vi "Registry-Based Logging (Wireless).vi"() -> ()   [LabVIEW 2018]
uses:
  api/logger_class/Log Levels.ctl
  api/logger_class/Failure Information.ctl
  api/logger_class/Log Record.ctl
  api/logger_class/Internal Log Levels.ctl
  ff44e4a9-c346-414c-ae2a-efcf3ff82913.vi
  968e9200-95f1-4d5c-ab7a-f172df11adbb.vi
  5746b3ac-eb64-4ad0-8e88-1d5da43a9e78.vi
  ee222f89-d58e-4e28-8b53-aa2841b98c47.vi
  645936a5-18e5-41ae-9078-b5e4c552694f.vi
  c7798b5a-73a1-416c-972e-a12d59322e34.vi
  1f8b4f84-eef8-41cb-aaa5-2323aa4fe3ca.vi
  b5f8ac20-1bad-4c30-9ea3-a10bb6eeb7f6.vi
  968e9200-95f1-4d5c-ab7a-f172df11adbb.vi/caf2d4a3-5a7b-40e1-b7b0-74b52901b9f9.vi
  5746b3ac-eb64-4ad0-8e88-1d5da43a9e78.vi/a02c6254-97f5-44e3-a3a9-7fdb6dfbd055.vi
  ee222f89-d58e-4e28-8b53-aa2841b98c47.vi/bae24b8d-f663-491e-8374-2218e527d0d0.vi
  api/Log.vi
  645936a5-18e5-41ae-9078-b5e4c552694f.vi/bf655d3c-1ce4-400f-a78f-0f3f0191886e.vi
  api/Mark Error.vi
  c7798b5a-73a1-416c-972e-a12d59322e34.vi/ba94d47b-0e30-4c32-b8ff-86d609cd95a5.vi
  968e9200-95f1-4d5c-ab7a-f172df11adbb.vi/caf2d4a3-5a7b-40e1-b7b0-74b52901b9f9.vi/0a1ee2ab-da6d-4243-8cf3-8125e611a602.vi
  5746b3ac-eb64-4ad0-8e88-1d5da43a9e78.vi/a02c6254-97f5-44e3-a3a9-7fdb6dfbd055.vi/73f0ec31-6bdf-4568-9d3b-fef50ac01b30.vi
  ee222f89-d58e-4e28-8b53-aa2841b98c47.vi/bae24b8d-f663-491e-8374-2218e527d0d0.vi/6f202c45-f0ca-42f4-9f63-a87d9fe0c32d.vi
  api/configuration/handlers/string_handler/String Handler.lvclass
  C:/Users/Colin/Documents/software_projects/labview/glog/src/api/extension/formatting_handler_interface/Formatting Handler.lvclass
  api/configuration/formatters/JSON_formatter/JSON.lvclass
  C:/Users/Colin/Documents/software_projects/labview/glog/src/api/extension/formatter_interface/Formatter.lvclass
  <vilib>/Utility/error.llb/Error Cluster From Error Code.vi
  registry/Enable All.vi
  registry/Disable All.vi
  registry/Log.vi
  <vilib>/ErrorRing/Error Ring.xnode
  api/GLog.lvlib
  api/logger_class/Logger.lvclass
panel:
  out "total time [ms]":u32
  out "logging time [ms]":u32
  in  "Failure Type":bool
  out "failures info":T1[](array[typedef]) {"Log Record"."timestamp" format="%<%x %.3X>T"}
  in  "error/warning iteration":i32=20
  in  "log messages 2":string
  in  "loop iteration delay [ms]":u32=10
  in  "minimum log level":T4=enum."Info"
  out "error out":errorcluster
  in  "log messages":string
  in  "total iterations":i32=30
  in  "restart logging at":i32=20
  in  "stop logging at":i32=10
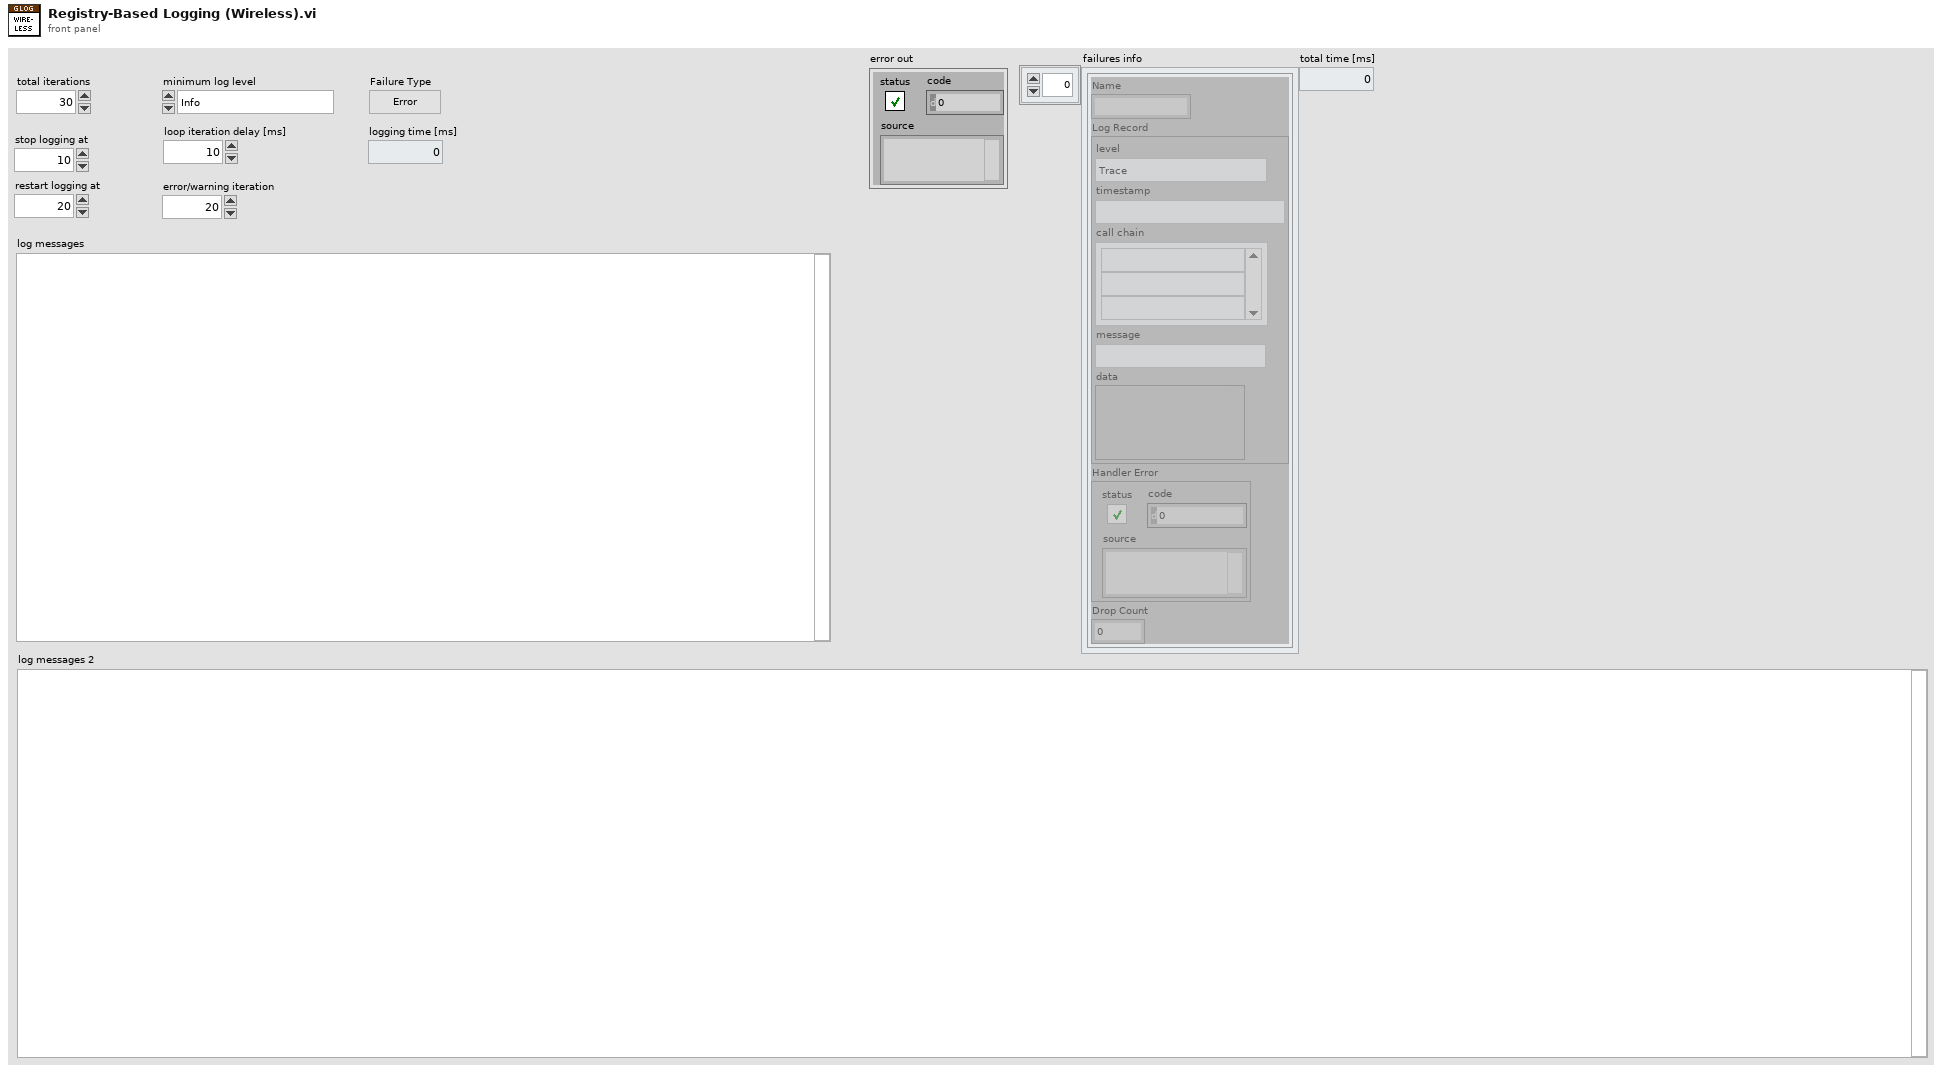
[diagram p1: front panel]
types:
  T1 = typedef "GLog.lvlib/Logger.lvclass/Failure Information.ctl" = cluster{"Name":string, "Log Record":T2, "Handler Error":errorcluster, "Drop Count":u32}
  T2 = typedef "GLog.lvlib/Logger.lvclass/Log Record.ctl" = cluster{"level":T3, "timestamp":timestamp, "call chain":string[], "message":string, "data":variant}
  T3 = typedef "GLog.lvlib/Logger.lvclass/Internal Log Levels.ctl" = enum16{"Trace", "Debug", "Info", "Warning", "Error", "Critical", "Internal"}
  T4 = typedef "GLog.lvlib/Logger.lvclass/Log Levels.ctl" = enum16{"Trace", "Debug", "Info", "Warning", "Error", "Critical"}
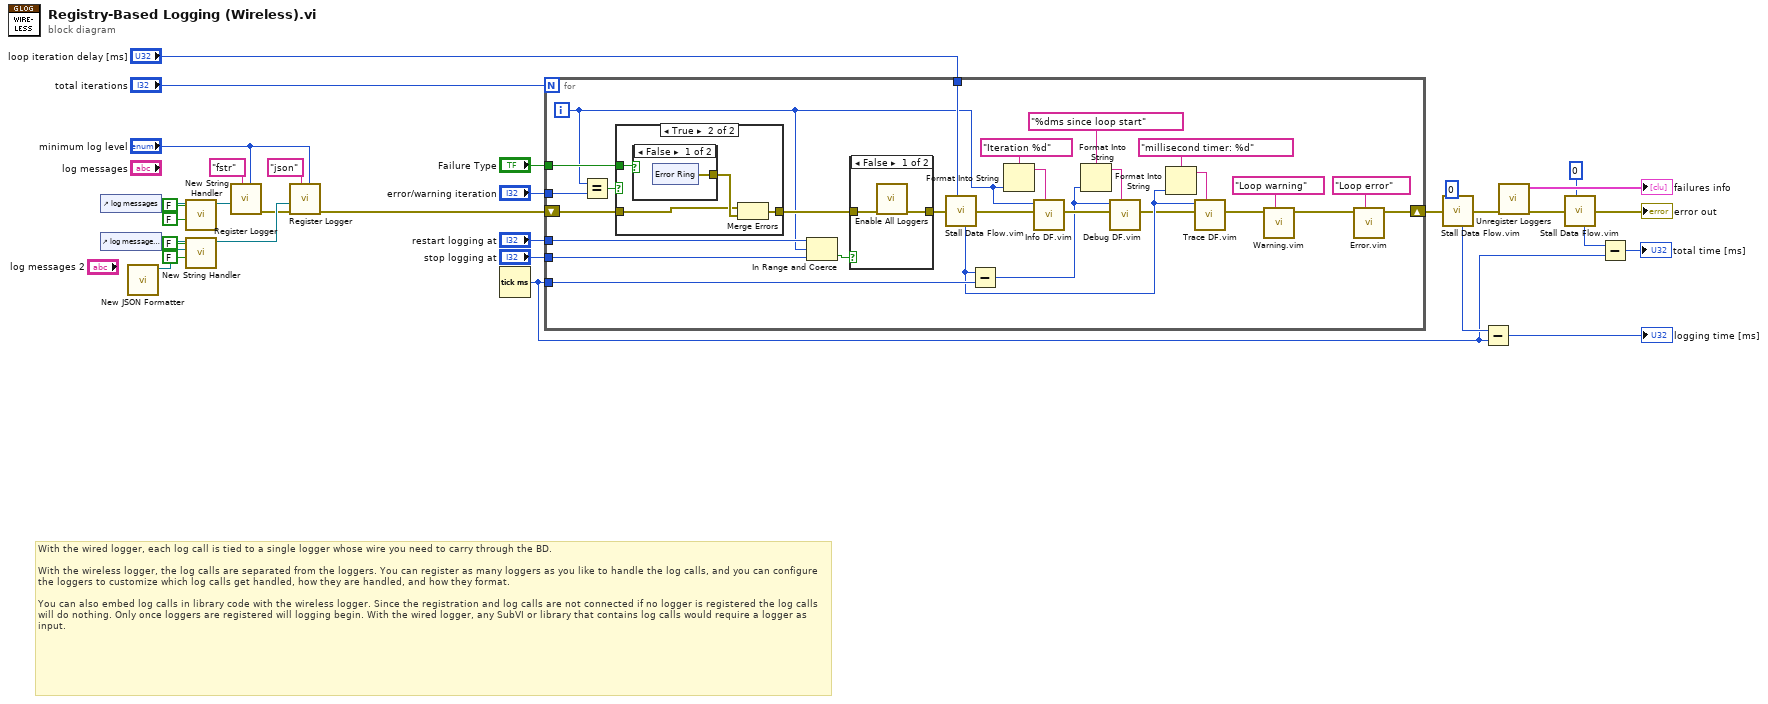
[diagram p0: block diagram]
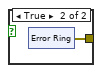
[diagram p3: hidden frame]
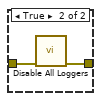
[diagram p4: hidden frame]
diagram:
  # "With the wired logger, each log call is tied to a single logger whose wire you need to carry through the BD.\n\nWith the wireless logger, the log calls are separated from the loggers. You can register as many loggers as you like to handle the log calls, and you can configure the loggers to customize which log calls get handled, how they are handled, and how they format.\n\nYou can also embed log calls in library code with the wireless logger. Since the registration and log calls are not connected if no logger is registered the log calls will do nothing. Only once loggers are registered will logging begin. With the wired logger, any SubVI or library that contains log calls would require a logger as input."
  n1 = control-ref of="log messages"() -> (w28:refnum<vi>)
  n2 = control-ref of="log messages 2"() -> (w25:refnum<vi>)
  n3 = call "New JSON Formatter.vi"() -> ("JSON formatter"=w23:refnum<class "JSON.lvclass">)  [unwired: 11 in]
  n4 = call "New String Handler.vi"("auto-scroll? (T)"=FALSE, "multi-line? (T)"=FALSE, "string control"=w28) -> ("new string handler"=w29:refnum<class "String Handler.lvclass">)  [unwired: 8 in]
  n5 = call "New String Handler.vi"("auto-scroll? (T)"=FALSE, "multi-line? (T)"=FALSE, "formatter (format string)"=w23, "string control"=w25) -> ("new string handler"=w24:refnum<class "String Handler.lvclass">)  [unwired: 7 in]
  n6 = call "Register Logger.vi"("minimum log level (Info)"="minimum log level", "name (\"Default\")"="fstr" ("name (\"Default\")"), "log handler (file handler)"=w29) -> ("error out"=w17:errorcluster)  [unwired: 8 in]
  n7 = call "Register Logger.vi"("minimum log level (Info)"="minimum log level", "name (\"Default\")"="json" ("name (\"Default\")"), "error in (no error)"=w17, "log handler (file handler)"=w24) -> ("error out"=w16:errorcluster)  [unwired: 7 in]
  n8 = Tick Count (ms)() -> (millisecond timer value=w5:u32)
  n9 = for {
    N: "total iterations" -> [_]
    tunnel: w5 -> [w60]
    tunnel: "stop logging at" -> [w58]
    tunnel: "restart logging at" -> [w57]
    shift-right: [w43] -> w14
    shift-left: w16 -> [w39]
    tunnel: "loop iteration delay [ms]" -> [w55]
    tunnel: "error/warning iteration" -> [w41]
    tunnel: "Failure Type" -> [w34]
    i -> [w33]
    n10 = Equal?(x=w33, y=w41) -> (x = y?=w40:bool)
    n11 = case shown="True" w40 {
      tunnel: w39 -> [w61 w63]
      tunnel: [w61 w64] -> w38
      tunnel: w34 -> [_ w62]
      frame False {
      }
      frame True {
        n12 = case shown="False" w62 {
          tunnel: [w66 w72] -> w65
          frame False {
            n13 = xnode "Error Ring"() -> ("error out"=w66:errorcluster)
          }
          frame True {
            n14 = xnode "Error Ring"() -> ("error out"=w72:errorcluster)
          }
        }
        n15 = Merge Errors(w63, w65) -> (w64:errorcluster)
      }
    }
    n16 = In Range and Coerce(upper limit=w57, x=w33, lower limit=w58) -> (In Range?=w59:bool)  [unwired: 1 out]
    n17 = case shown="False" w59 {
      tunnel: w38 -> [w79 w81]
      tunnel: [w78 w80] -> w54
      frame False {
        n18 = call "Enable All Loggers.vi"("error in"=w79) -> ("error out"=w78:errorcluster)  [unwired: 10 in]
      }
      frame True {
        n19 = call "Disable All Loggers.vi"("error in"=w81) -> ("error out"=w80:errorcluster)  [unwired: 10 in]
      }
    }
    n20 = call "Stall Data Flow.vim"("value in"=w54, "milliseconds to wait"=w55) -> ("millisecond timer value"=w45:u32, "value out"=w53:errorcluster)
    n21 = Subtract(x=w45, y=w60) -> (x-y=w49:u32)
    n22 = Format Into String(format string="Iteration %d" ("message"), w33) -> (resulting string=w52:string)  [unwired: 2 in, 1 out]
    n23 = call "Info DF.vim"("message"=w52, "dataflow in"=w53, "data (null)"=w33) -> ("dataflow out"=w50:errorcluster)  [unwired: 8 in]
    n24 = Format Into String(format string="%dms since loop start" ("message"), w49) -> (resulting string=w51:string)  [unwired: 2 in, 1 out]
    n25 = call "Debug DF.vim"("message"=w51, "dataflow in"=w50, "data (null)"=w49) -> ("dataflow out"=w44:errorcluster)  [unwired: 8 in]
    n26 = Format Into String(format string="millisecond timer: %d" ("message"), w45) -> (resulting string=w46:string)  [unwired: 2 in, 1 out]
    n27 = call "Trace DF.vim"("message"=w46, "dataflow in"=w44, "data (null)"=w45) -> ("dataflow out"=w37:errorcluster)  [unwired: 8 in]
    n28 = call "Warning.vim"("data in (null)"=w37, "message"="Loop warning") -> ("data out"=w36:errorcluster)  [unwired: 9 in]
    n29 = call "Error.vim"("data in (null)"=w36, "message"="Loop error") -> ("data out"=w43:errorcluster)  [unwired: 9 in]
  }
  n30 = call "Stall Data Flow.vim"("value in"=w14, "milliseconds to wait"=u32 0) -> ("millisecond timer value"=w12:u32, "value out"=w13:errorcluster)
  n31 = Subtract(x=w12, y=w5) -> (x-y=→"logging time [ms]":u32)
  n32 = call "Unregister Loggers.vi"("error in (no error)"=w13) -> ("error out"=w26:errorcluster, "failures info"=→"failures info":T1[])  [unwired: 9 in]
  n33 = call "Stall Data Flow.vim"("value in"=w26, "milliseconds to wait"=u32 0) -> ("millisecond timer value"=w6:u32, "value out"=→"error out":errorcluster)
  n34 = Subtract(x=w6, y=w5) -> (x-y=→"total time [ms]":u32)
